vi "Create Point Channels.vi"(8 "error in (no error)":errorcluster, 9 "adv_para":i32, 10 "PlayerID":u8, 11 "Parent Ref in":T1 format="%.0x") -> (0 "error out":errorcluster, 3 "Parent Ref out":T1=18446744073709551615 format="%.0x")   [LabVIEW 2023, in "Vires VTD System Explorer.lvlib"]
uses:
  Vires VTD System Explorer.lvlib
  <vilib>/NI VeriStand/Custom Device API/Custom Device Item Ref.ctl
  <vilib>/NI VeriStand/Custom Device API/Custom Device Channel.ctl
  <vilib>/NI VeriStand/Custom Device API/Custom Device Channel Type.ctl
  <vilib>/xnet/xnet.llb/XNET String To IO Name (Frame).vi
  <resource>/objmgr/xnet.rc
  <vilib>/NI VeriStand/Custom Device API/Custom Device API.lvlib
panel:
  out "Name (Short)":string
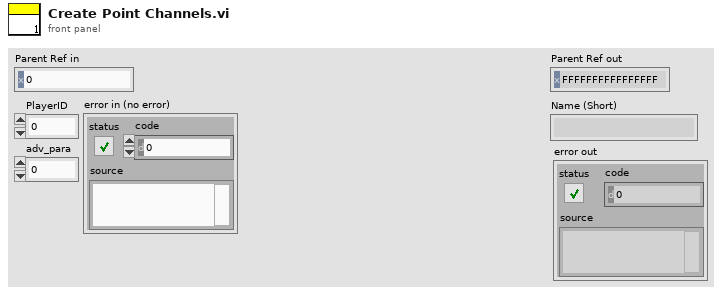
[diagram p1: front panel]
types:
  T1 = typedef "Custom Device API.lvlib/Custom Device Item Ref.ctl" = u64
  T2 = typedef "Custom Device API.lvlib/Custom Device Channel.ctl" = cluster{"Type":T3, "Units":string, "Default Value":dbl, "Faultable":bool, "Scalable":bool}
  T3 = typedef "Custom Device API.lvlib/Custom Device Channel Type.ctl" = enum16{"Input", "Output"}
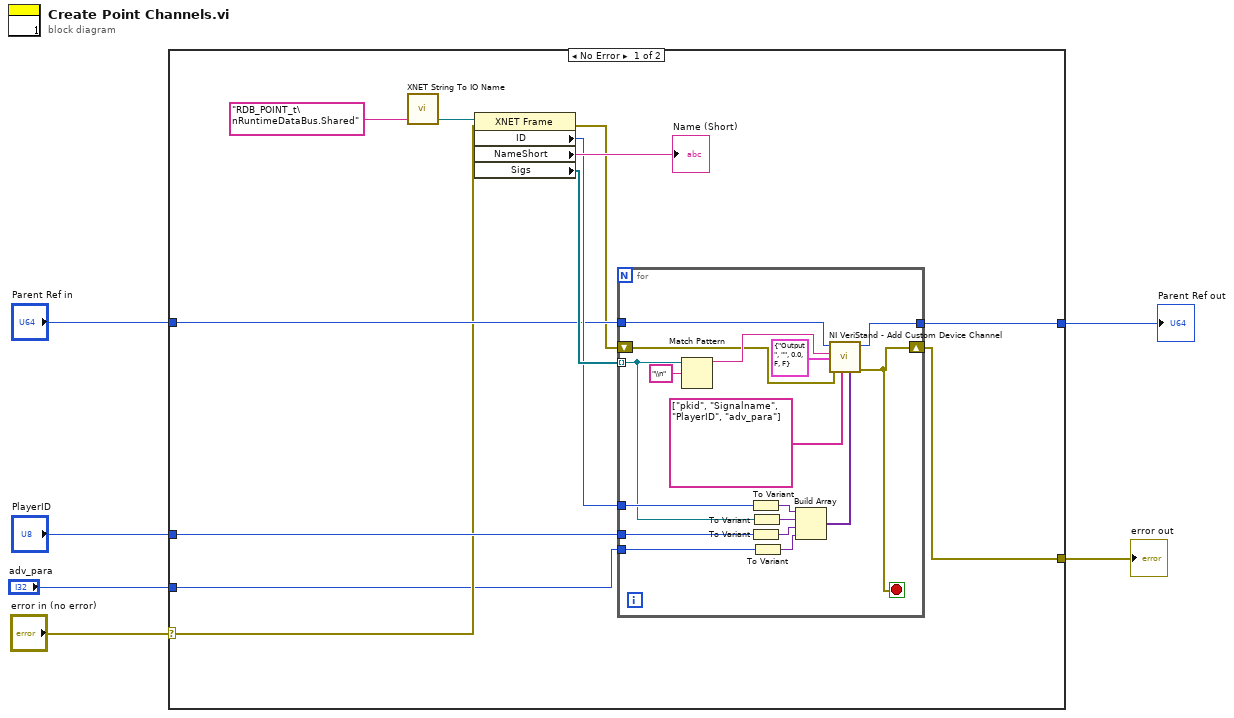
[diagram p0: block diagram]
diagram:
  n1 = case shown="No Error" "error in (no error)" {
    selector: "error in (no error)" -> [w10 w37]
    tunnel: "Parent Ref in" -> [w13 w36]
    tunnel: [w12 w36] -> w5
    tunnel: "PlayerID" -> [w11 _]
    tunnel: [w8 w37] -> w2
    tunnel: "adv_para" -> [w7 _]
    frame No Error {
      n2 = call-poly <vilib>:"XNET String To IO Name.vi"("string"="RDB_POINT_t\nRuntimeDataBus.Shared") -> ("XNET Frame"=w15:refnum<k21>)  [unwired: 4 out]
      n3 = property class="XNET Frame"(reference=w15, error in=w10) -> (error out=w9:errorcluster, "ID"=w14:u32, "NameShort"=→"Name (Short)":string, "Sigs"=w17:refnum<k21>[])  [unwired: 1 out]
      n4 = for {
        tunnel: w17 -> [w26] mode=indexing
        tunnel: w14 -> [w27]
        tunnel: w13 -> [w24]
        tunnel: [w23] -> w12
        tunnel: w11 -> [w22]
        shift-right: [w20] -> w8
        shift-left: w9 -> [w21]
        tunnel: w7 -> [w19]
        stop <- w20 stop-if-true
        n5 = Match Pattern(string=w26, regular expression="\\n") -> (before substring=w25:string)  [unwired: 1 in, 3 out]
        n6 = To Variant(anything=w27) -> (Variant=w33:variant)
        n7 = To Variant(anything=w22) -> (Variant=w32:variant)
        n8 = To Variant(anything=w26) -> (Variant=w30:variant)
        n9 = To Variant(anything=w19) -> (Variant=w34:variant)
        n10 = Build Array(w33, w30, w32, w34) -> (w31:variant[])
        n11 = call <vilib>:"NI VeriStand - Add Custom Device Channel.vi"("Property Values"=w31, "Property names"=string[] ["pkid", "Signalname", "PlayerID", "adv_para"], "error in (no error)"=w21, "Channel"=T2 {"Type"=enum."Output", "Units"="", "Default Value"=0.0, "Faultable"=FALSE, "Scalable"=FALSE}, "Channel Name"=w25, "Parent Ref in"=w24) -> ("error out"=w20:errorcluster, "Parent Ref out"=w23:T1)  [unwired: 2 in, 2 out]
      }
    }
    frame Error {
    }
  }
  "Parent Ref out" <- w5
  "error out" <- w2
